vi "Load Sequence.vi"(6 "Fallback Name":string, 7 "CRC":u32 format="%08x", 8 "error in (no error)":refnum<class "MultiErrors.lvclass">, 10 "Config Element":refnum<class "Config Element.lvclass">) -> (0 "error out":refnum<class "MultiErrors.lvclass">, 3 "Sequence Config out":refnum<class "Sequence Config.lvclass">)   [LabVIEW 2023, in "VolatusSeqConfig.lvlib" / "Sequence Config.lvclass"]
uses:
  Sequence Config.lvclass
  VolatusErrorUtilities/MultiErrors/MultiErrors.lvclass
  lv-cdm/CDM-Config/Config Element/Config Element.lvclass
  Debug Flags.ctl
  VolatusErrorUtilities/MultiErrors/MultiErrors.lvclass/MultiErrors.ctl
  Sequence Config.lvclass/Sequence Config.ctl
  Sequence Constants/Sequence Constants.lvclass
  VolatusSeqConfig.lvlib
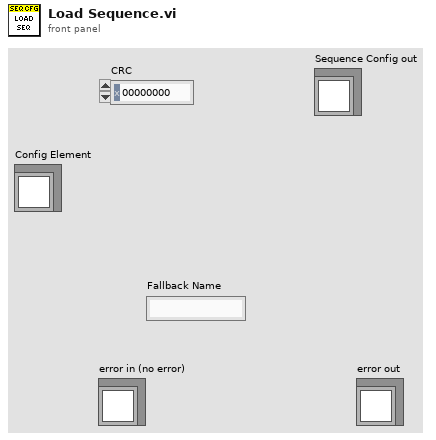
[diagram p1: front panel]
types:
  T1 = typedef "VolatusSeqConfig.lvlib/Debug Flags.ctl" = cluster{"States":bool, "Conditions":bool, "Timing":bool}
  T2 = typedef "VolatusSeqConfig.lvlib/Variable.ctl" = cluster{"Name":string, "Value":dbl, "Comment":string}
  T3 = typedef "VolatusSeqConfig.lvlib/State.ctl" = cluster{"Name":string, "Steps":T4[], "Transitions":refnum<class "Transition Config.lvclass">[], "Comment":string, "Color":string, "Seq Name":string, "Debug":T1}
  T4 = typedef "VolatusSeqConfig.lvlib/Step.ctl" = cluster{"Time":dbl, "Commands":refnum<class "Command Config.lvclass">[]}
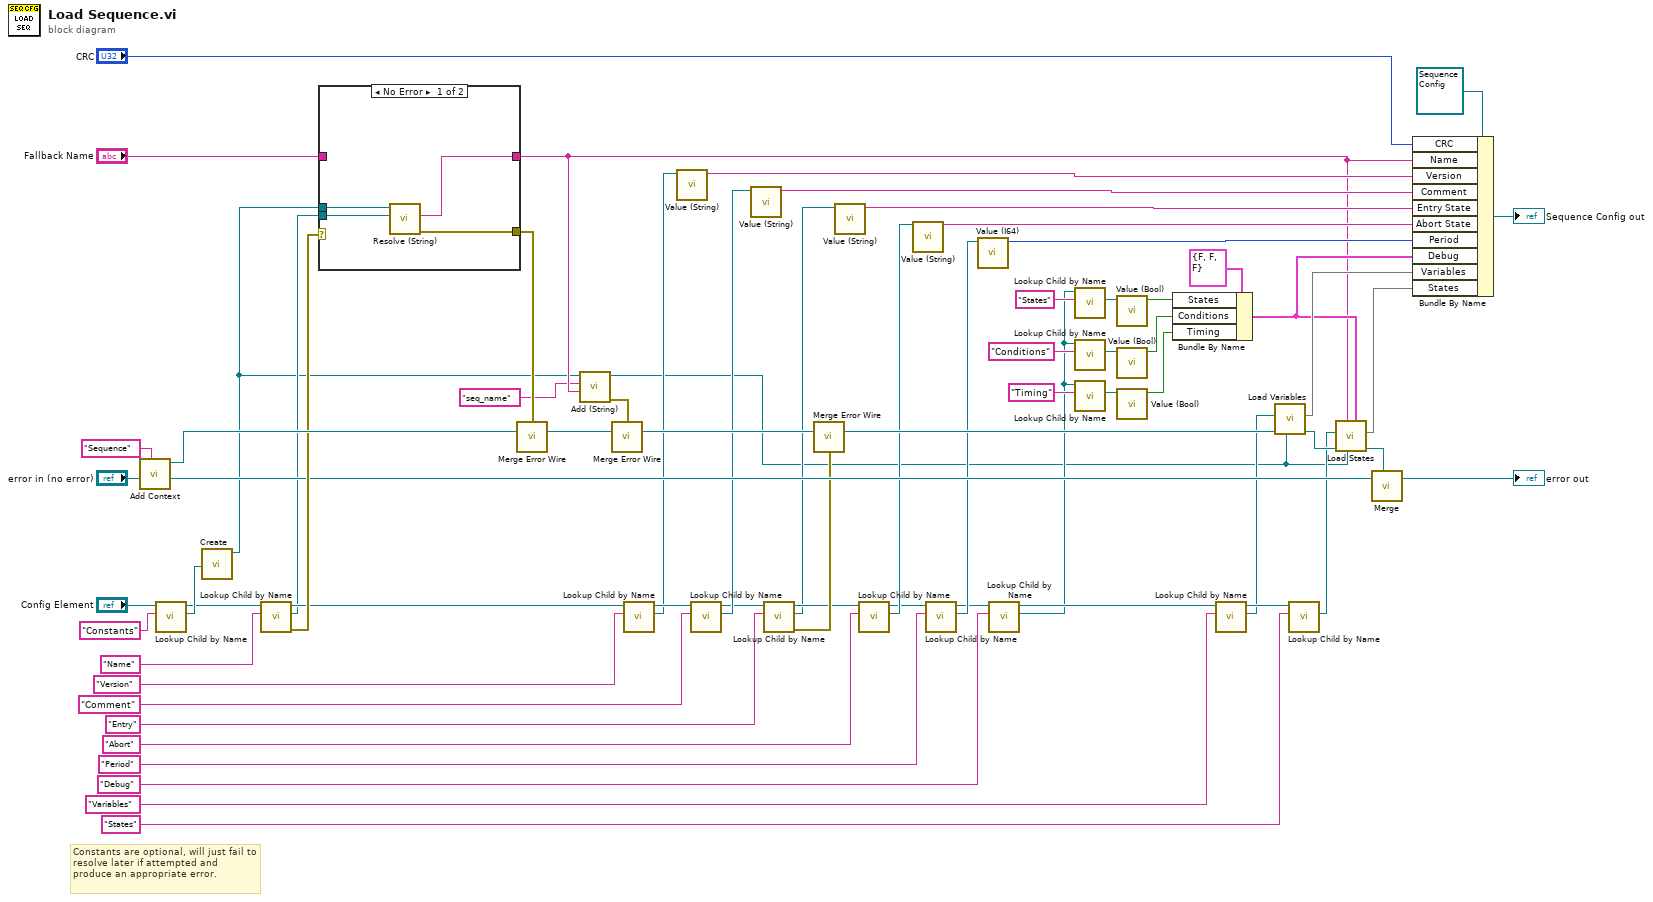
[diagram p0: block diagram]
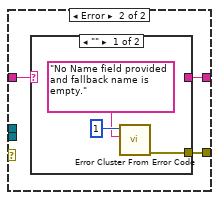
[diagram p2: hidden frame]
diagram:
  # "Constants are optional, will just fail to resolve later if attempted and produce an appropriate error."
  n1 = call "Add Context.vi"("Context"="Sequence", "MultiErrors in"="error in (no error)") -> ("Original Context"=w67:refnum<class "MultiErrors.lvclass">, "Added Context"=w69:refnum<class "MultiErrors.lvclass">)  [unwired: 8 in]
  n2 = call "Lookup Child by Name.vi"("Name"="Constants", "Config Element in"="Config Element") -> ("Child"=w26:refnum<class "Config Element.lvclass">, "Config Element out"=w15:refnum<class "Config Element.lvclass">)  [unwired: 6 in, 2 out]
  n3 = call "Create.vi"("Element"=w26) -> ("Sequence Constants out"=w5:refnum<class "Sequence Constants.lvclass">)  [unwired: 9 in, 1 out]
  n4 = call "Lookup Child by Name.vi"("Name"="Name", "Config Element in"=w15) -> ("error out"=w68:errorcluster, "Child"=w36:refnum<class "Config Element.lvclass">, "Config Element out"=w61:refnum<class "Config Element.lvclass">)  [unwired: 6 in, 1 out]
  n5 = case shown="No Error" w68 {
    tunnel: w36 -> [w74 _]
    tunnel: [w73 w76] -> w6
    tunnel: w5 -> [w72 _]
    tunnel: "Fallback Name" -> [_ w77]
    tunnel: [w71 w75] -> w12
    frame No Error {
      n6 = call "Resolve (String).vi"("Element"=w74, "Sequence Constants in"=w72) -> ("error out"=w71:errorcluster, "String Value"=w73:string)  [unwired: 7 in, 1 out]
    }
    frame Error {
      n7 = case shown="\"\"" w77 {
        selector: w77 -> [_ w81]
        tunnel: [_ w81] -> w76
        tunnel: [w78 _] -> w75
        frame "" {
          n8 = call <vilib>:"Error Cluster From Error Code.vi"("error message (\"\")"="No Name field provided and fallback name is empty.", "error code (0)"=1) -> ("error out"=w78:errorcluster)  [unwired: 7 in]
        }
        frame Default {
        }
      }
    }
  }
  n9 = call "Merge Error Wire.vi"("error in (no error)"=w12, "MultiErrors in"=w69) -> ("MultiErrors out"=w3:refnum<class "MultiErrors.lvclass">)  [unwired: 13 in]
  n10 = call "Add (String).vi"("Value"=w6, "Name"="seq_name", "Sequence Constants in"=w5) -> ("error out"=w2:errorcluster, "Sequence Constants out"=w4:refnum<class "Sequence Constants.lvclass">)  [unwired: 7 in]
  n11 = call "Merge Error Wire.vi"("error in (no error)"=w2, "MultiErrors in"=w3) -> ("MultiErrors out"=w70:refnum<class "MultiErrors.lvclass">)  [unwired: 13 in]
  n12 = call "Lookup Child by Name.vi"("Name"="Version", "Config Element in"=w61) -> ("Child"=w52:refnum<class "Config Element.lvclass">, "Config Element out"=w59:refnum<class "Config Element.lvclass">)  [unwired: 6 in, 2 out]
  n13 = call "Value (String).vi"("Config Element in"=w52) -> ("String Value"=w51:string)  [unwired: 9 in, 1 out]
  n14 = call "Lookup Child by Name.vi"("Name"="Comment", "Config Element in"=w59) -> ("Child"=w50:refnum<class "Config Element.lvclass">, "Config Element out"=w38:refnum<class "Config Element.lvclass">)  [unwired: 6 in, 2 out]
  n15 = call "Value (String).vi"("Config Element in"=w50) -> ("String Value"=w49:string)  [unwired: 9 in, 1 out]
  n16 = call "Lookup Child by Name.vi"("Name"="Entry", "Config Element in"=w38) -> ("error out"=w66:errorcluster, "Child"=w43:refnum<class "Config Element.lvclass">, "Config Element out"=w44:refnum<class "Config Element.lvclass">)  [unwired: 6 in, 1 out]
  n17 = call "Merge Error Wire.vi"("error in (no error)"=w66, "MultiErrors in"=w70) -> ("MultiErrors out"=w65:refnum<class "MultiErrors.lvclass">)  [unwired: 13 in]
  n18 = call "Value (String).vi"("Config Element in"=w43) -> ("String Value"=w40:string)  [unwired: 9 in, 1 out]
  n19 = call "Lookup Child by Name.vi"("Name"="Abort", "Config Element in"=w44) -> ("Child"=w41:refnum<class "Config Element.lvclass">, "Config Element out"=w31:refnum<class "Config Element.lvclass">)  [unwired: 6 in, 2 out]
  n20 = call "Value (String).vi"("Config Element in"=w41) -> ("String Value"=w39:string)  [unwired: 9 in, 1 out]
  n21 = call "Lookup Child by Name.vi"("Name"="Period", "Config Element in"=w31) -> ("Child"=w28:refnum<class "Config Element.lvclass">, "Config Element out"=w25:refnum<class "Config Element.lvclass">)  [unwired: 6 in, 2 out]
  n22 = call "Value (I64).vi"("Config Element in"=w28) -> ("I64 Value"=w29:i64)  [unwired: 9 in, 1 out]
  n23 = call "Lookup Child by Name.vi"("Name"="Debug", "Config Element in"=w25) -> ("Child"=w9:refnum<class "Config Element.lvclass">, "Config Element out"=w14:refnum<class "Config Element.lvclass">)  [unwired: 6 in, 2 out]
  n24 = call "Lookup Child by Name.vi"("Name"="States", "Config Element in"=w9) -> ("Child"=w20:refnum<class "Config Element.lvclass">)  [unwired: 6 in, 3 out]
  n25 = call "Lookup Child by Name.vi"("Name"="Conditions", "Config Element in"=w9) -> ("Child"=w18:refnum<class "Config Element.lvclass">)  [unwired: 6 in, 3 out]
  n26 = call "Lookup Child by Name.vi"("Name"="Timing", "Config Element in"=w9) -> ("Child"=w11:refnum<class "Config Element.lvclass">)  [unwired: 6 in, 3 out]
  n27 = call "Value (Bool).vi"("Config Element in"=w20) -> ("Bool Value"=w19:bool)  [unwired: 9 in, 1 out]
  n28 = call "Value (Bool).vi"("Config Element in"=w18) -> ("Bool Value"=w17:bool)  [unwired: 9 in, 1 out]
  n29 = call "Value (Bool).vi"("Config Element in"=w11) -> ("Bool Value"=w8:bool)  [unwired: 9 in, 1 out]
  n30 = Bundle By Name(cluster=T1 {"States"=FALSE, "Conditions"=FALSE, "Timing"=FALSE} ("Events"), "States"=w19, "Conditions"=w17, "Timing"=w8) -> (w7:T1)
  n31 = call "Lookup Child by Name.vi"("Name"="Variables", "Config Element in"=w14) -> ("Child"=w54:refnum<class "Config Element.lvclass">, "Config Element out"=w56:refnum<class "Config Element.lvclass">)  [unwired: 6 in, 2 out]
  n32 = call "Load Variables.vi"("Constants"=w4, "error in (no error)"=w65, "Config Element"=w54) -> ("error out"=w64:refnum<class "MultiErrors.lvclass">, "Variables"=w48:map{string, T2})  [unwired: 7 in]
  n33 = call "Lookup Child by Name.vi"("Name"="States", "Config Element in"=w56) -> ("Child"=w47:refnum<class "Config Element.lvclass">)  [unwired: 6 in, 3 out]
  n34 = call "Load States.vi"("Debug"=w7, "Constants"=w4, "Seq Name"=w6, "error in"=w64, "Config Element"=w47) -> ("error out"=w33:refnum<class "MultiErrors.lvclass">, "States"=w46:map{string, T3})  [unwired: 5 in]
  n35 = call "Merge.vi"("First Error In"=w67, "Second Error In"=w33) -> ("MultiErrors out"=→"error out":refnum<class "MultiErrors.lvclass">)  [unwired: 5 in]
  n36 = Bundle By Name(cluster=refnum<class "Sequence Config.lvclass"> refnum ("Sequence Config in"), "CRC"="CRC", "Name"=w6, "Version"=w51, "Comment"=w49, "Entry State"=w40, "Abort State"=w39, "Period"=w29, "Debug"=w7, "Variables"=w48, "States"=w46) -> (→"Sequence Config out":refnum<class "Sequence Config.lvclass">)
